vi "Change Database.vi"(8 "error in (no error)":errorcluster, 11 "Node Ptr":u64 format="%.0x") -> (0 "error out":errorcluster)   [LabVIEW 2025, in "Protection and Counter Addon System Explorer.lvlib"]
uses:
  Protection and Counter Addon System Explorer.lvlib
  Types/Database Changes VS Existing Frames.ctl
  Types/Base Frame Info.ctl
  <vilib>/NI VeriStand/Custom Device API/Custom Device Item Ref.ctl
  Types/CAN Filter Type.ctl
  Addon Shared/SubVIs/GUID Lookup.vi
  <vilib>/NI/NI VeriStand Advanced SysDef API/_SubVIs/SysDef.Search.GUIDs.vi
  <vilib>/NI VeriStand/Custom Device API/Get Item Property (U32).vi
  Addon Shared/Protection and Counter Addon Shared.lvlib
  <vilib>/NI/NI VeriStand Advanced SysDef API/SysDef API/Advanced System Definition.lvlib
  <vilib>/NI VeriStand/Custom Device API/Custom Device API.lvlib
  <resource>/objmgr/xnet.rc
  <vilib>/NI VeriStand/Custom Device Tools/Custom Device Utility Library/Custom Device Utility Library.lvlib
panel:
  in  "Tag":string
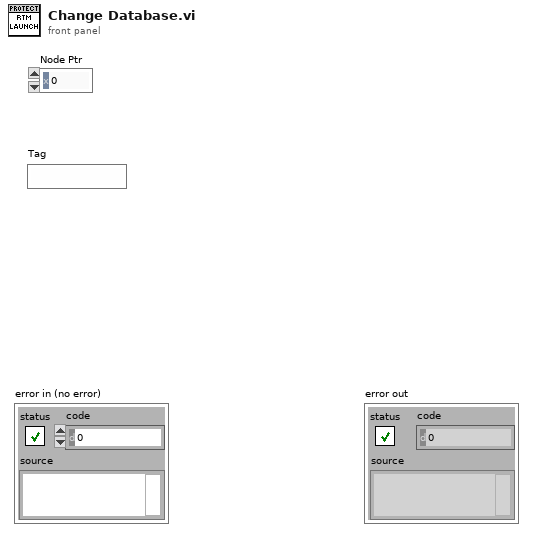
[diagram p1: front panel]
types:
  T1 = typedef "Protection and Counter Addon System Explorer.lvlib/Database Changes VS Existing Frames.ctl" = cluster{"Incoming":T2[], "Outgoing":T2[]}
  T2 = typedef "Protection and Counter Addon System Explorer.lvlib/Base Frame Info.ctl" = cluster{"Name":string, "ID":u32, "Signals":string[], "Node Ref":T3, "Type":T4}
  T3 = typedef "Custom Device API.lvlib/Custom Device Item Ref.ctl" = u64
  T4 = typedef "Protection and Counter Addon System Explorer.lvlib/CAN Filter Type.ctl" = enum16{"Cyclic Data", "Event Data", "Cyclic/Event", "All"}
  T5 = typedef "Custom Device API.lvlib/Custom Device Item Info.ctl" = cluster{"Name":string, "Is Channel":bool, "GUID":string, "Is Waveform":bool}
  T6 = typedef "Protection and Counter Addon Shared.lvlib/XNET Settings.ctl" = cluster{"Database":refnum<k21>, "Cluster":refnum<k21>, "Port":string, "Baud rate [Bd]":u64, "Termination":u32, "CAN I/O Mode":u32, "FD Baud rate [Bd]":u64, "Priority":i32, "Use Legacy":bool, "FD ISO Mode":u32, "Default Max Counter Value":dbl, "Default Protect Type":T7, "Include All Channels":bool}
  T7 = typedef "Protection and Counter Support Shared.lvlib/Protection Type.ctl" = enum16{"Arb ID + Bytes Checksum with Inversion", "Arb ID + Bytes CRC with Inversion", "Reversed Raw Signal Checksum with Inversion", "Concatenated Two's Compliment"}
  T8 = typedef "Protection and Counter Addon System Explorer.lvlib/CAN Update Results.ctl" = cluster{"New Cluster":refnum<k21>, "Incoming":T9, "Outgoing":T9}
  T9 = typedef "Protection and Counter Addon System Explorer.lvlib/VS Update List.ctl" = cluster{"Frames to Delete":T3[], "Frames to Add":T10[], "Frames to Update":T12[]}
  T10 = typedef "Protection and Counter Addon System Explorer.lvlib/Base Frame Info_NoVS.ctl" = cluster{"Name":string, "ID":u32, "Signals":T11[], "Type":T4}
  T11 = typedef "Protection and Counter Addon System Explorer.lvlib/Signal Attributes.ctl" = cluster{"Name":string, "Value Table":string, "Units":string}
  T12 = typedef "Protection and Counter Addon System Explorer.lvlib/CAN Frame Update Results.ctl" = cluster{"Node Ref":T3, "Name":string, "ID":u32, "New Signals":T11[], "Delete Signals":string[], "Type":T4, "Update Signals":T11[]}
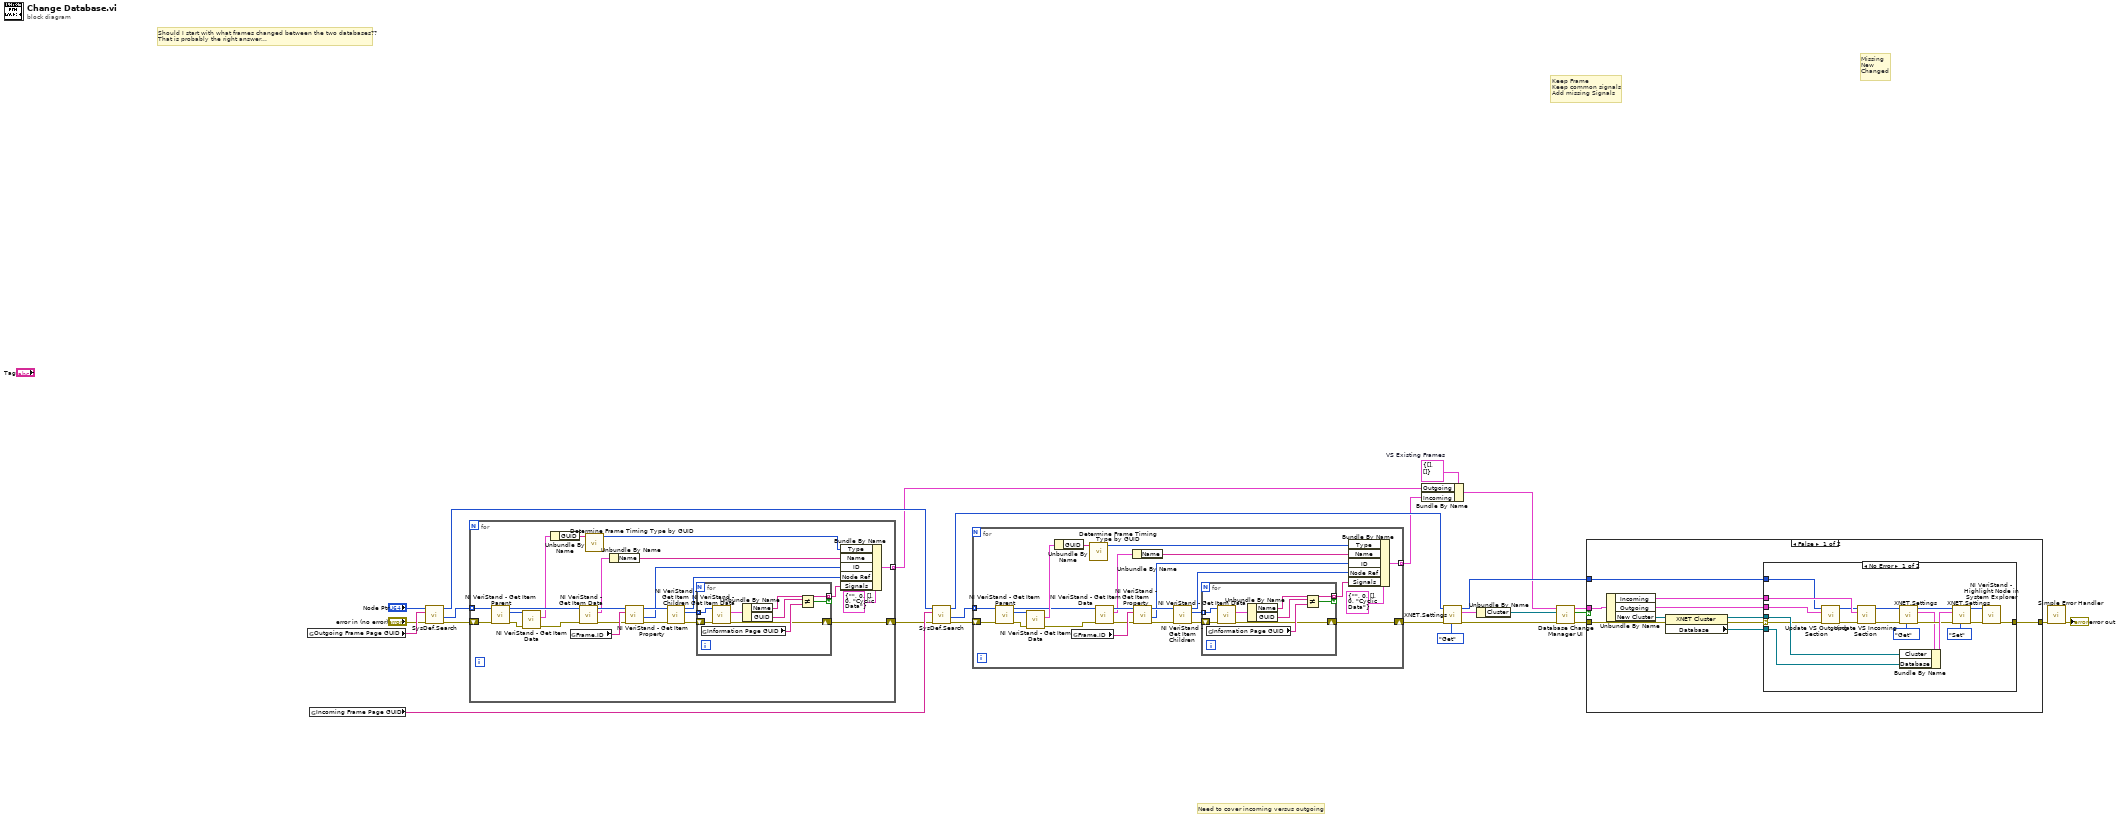
[diagram p0: block diagram]
diagram:
  w2 = T1 {"Incoming"=[], "Outgoing"=[]}  # VS Existing Frames
  # "Missing\nNew\nChanged"
  # "Should I start with what frames changed between the two databases??\nThat is probably the right answer..."
  # "Keep Frame\nKeep common signals\nAdd missing Signals"
  # "Need to cover incoming versus outgoing"
  n1 = global read "GUID Lookup.vi" "Outgoing Frame Page GUID"() -> (w26:string)
  n2 = global read "GUID Lookup.vi" "Incoming Frame Page GUID"() -> (w25:string)
  n3 = call-poly <vilib>:"SysDef.Search.vi"("error in (no error)"="error in (no error)", "GUID"=w26, "nodeID"="Node Ptr") -> ("error out"=w24:errorcluster, "Values Out"=w23:u64[], "nodeID out"=w19:u64)  [unwired: 5 in, 1 out]
  n4 = for {
    tunnel: w23 -> [w34] mode=indexing
    tunnel: [w40] -> w4 mode=indexing
    shift-right: [w39] -> w20
    shift-left: w24 -> [w33]
    n5 = call <vilib>:"NI VeriStand - Get Item Parent.vi"("error in (no error)"=w33, "Item Ref in"=w34) -> ("error out"=w31:errorcluster, "Parent Ref"=w32:T3, "Item Ref out"=w35:T3)  [unwired: 6 in, 1 out]
    n6 = call <vilib>:"NI VeriStand - Get Item Data.vi"("error in (no error)"=w31, "Item Ref in"=w32) -> ("error out"=w30:errorcluster, "Item Info"=w29:T5)  [unwired: 6 in, 2 out]
    n7 = Unbundle By Name(w29) -> ("GUID"=w28:string)
    n8 = global read "GUID Lookup.vi" "Frame.ID"() -> (w48:string)
    n9 = call <vilib>:"NI VeriStand - Get Item Data.vi"("error in (no error)"=w30, "Item Ref in"=w35) -> ("error out"=w45:errorcluster, "Item Info"=w43:T5, "Item Ref out"=w44:T3)  [unwired: 6 in, 1 out]
    n10 = call "Determine Frame Timing Type by GUID.vi"("GUID"=w28) -> ("CAN:Frame Type"=w27:T4)  [unwired: 10 in]
    n11 = Unbundle By Name(w43) -> ("Name"=w37:string)
    n12 = call-poly <vilib>:"NI VeriStand - Get Item Property.vi"("error in (no error)"=w45, "Property Name"=w48, "Item Ref in"=w44) -> ("error out"=w49:errorcluster, "Value"=w42:u32, "Item Ref out"=w50:T3)  [unwired: 5 in, 1 out]
    n13 = call <vilib>:"NI VeriStand - Get Item Children.vi"("error in (no error)"=w49, "Item Ref in"=w50) -> ("error out"=w46:errorcluster, "Child Refs"=w47:T3[], "Item Ref out"=w36:T3)  [unwired: 6 in, 1 out]
    n14 = for {
      tunnel: w47 -> [w58] mode=indexing
      shift-right: [w53] -> w39
      shift-left: w46 -> [w57]
      tunnel: [w51] -> w41 mode=indexing if=w52
      n15 = global read "GUID Lookup.vi" "Information Page GUID"() -> (w55:string)
      n16 = call <vilib>:"NI VeriStand - Get Item Data.vi"("error in (no error)"=w57, "Item Ref in"=w58) -> ("error out"=w53:errorcluster, "Item Info"=w56:T5)  [unwired: 6 in, 2 out]
      n17 = Unbundle By Name(w56) -> ("Name"=w51:string, "GUID"=w54:string)
      n18 = Not Equal?(x=w54, y=w55) -> (x != y?=w52:bool)
    }
    n19 = Bundle By Name(cluster=T2 {"Name"="", "ID"=0, "Signals"=[], "Node Ref"=0, "Type"=enum."Cyclic Data"}, "Type"=w27, "Name"=w37, "ID"=w42, "Node Ref"=w36, "Signals"=w41) -> (w40:T2)
  }
  n20 = call-poly <vilib>:"SysDef.Search.vi"("error in (no error)"=w20, "GUID"=w25, "nodeID"=w19) -> ("error out"=w21:errorcluster, "Values Out"=w22:u64[], "nodeID out"=w11:u64)  [unwired: 5 in, 1 out]
  n21 = for {
    tunnel: w22 -> [w62] mode=indexing
    shift-right: [w71] -> w12
    shift-left: w21 -> [w63]
    tunnel: [w70] -> w3 mode=indexing
    n22 = call <vilib>:"NI VeriStand - Get Item Parent.vi"("error in (no error)"=w63, "Item Ref in"=w62) -> ("error out"=w66:errorcluster, "Parent Ref"=w67:T3, "Item Ref out"=w60:T3)  [unwired: 6 in, 1 out]
    n23 = call <vilib>:"NI VeriStand - Get Item Data.vi"("error in (no error)"=w66, "Item Ref in"=w67) -> ("error out"=w61:errorcluster, "Item Info"=w65:T5)  [unwired: 6 in, 2 out]
    n24 = Unbundle By Name(w65) -> ("GUID"=w64:string)
    n25 = global read "GUID Lookup.vi" "Frame.ID"() -> (w80:string)
    n26 = call "Determine Frame Timing Type by GUID.vi"("GUID"=w64) -> ("CAN:Frame Type"=w59:T4)  [unwired: 10 in]
    n27 = call <vilib>:"NI VeriStand - Get Item Data.vi"("error in (no error)"=w61, "Item Ref in"=w60) -> ("error out"=w79:errorcluster, "Item Info"=w73:T5, "Item Ref out"=w77:T3)  [unwired: 6 in, 1 out]
    n28 = Unbundle By Name(w73) -> ("Name"=w72:string)
    n29 = call-poly <vilib>:"NI VeriStand - Get Item Property.vi"("error in (no error)"=w79, "Property Name"=w80, "Item Ref in"=w77) -> ("error out"=w78:errorcluster, "Value"=w74:u32, "Item Ref out"=w76:T3)  [unwired: 5 in, 1 out]
    n30 = call <vilib>:"NI VeriStand - Get Item Children.vi"("error in (no error)"=w78, "Item Ref in"=w76) -> ("error out"=w81:errorcluster, "Child Refs"=w82:T3[], "Item Ref out"=w68:T3)  [unwired: 6 in, 1 out]
    n31 = for {
      tunnel: w82 -> [w90] mode=indexing
      shift-right: [w85] -> w71
      shift-left: w81 -> [w89]
      tunnel: [w83] -> w75 mode=indexing if=w84
      n32 = global read "GUID Lookup.vi" "Information Page GUID"() -> (w87:string)
      n33 = call <vilib>:"NI VeriStand - Get Item Data.vi"("error in (no error)"=w89, "Item Ref in"=w90) -> ("error out"=w85:errorcluster, "Item Info"=w88:T5)  [unwired: 6 in, 2 out]
      n34 = Unbundle By Name(w88) -> ("Name"=w83:string, "GUID"=w86:string)
      n35 = Not Equal?(x=w86, y=w87) -> (x != y?=w84:bool)
    }
    n36 = Bundle By Name(cluster=T2 {"Name"="", "ID"=0, "Signals"=[], "Node Ref"=0, "Type"=enum."Cyclic Data"}, "Type"=w59, "Name"=w72, "ID"=w74, "Node Ref"=w68, "Signals"=w75) -> (w70:T2)
  }
  n37 = Bundle By Name(cluster=w2, "Outgoing"=w4, "Incoming"=w3) -> (w1:T1)
  n38 = call "XNET.Settings.vi"("Action"=enum8{"Get", "Set"}."Get", "error in (no error)"=w12, "Parent Ref in"=w11) -> ("error out"=w9:errorcluster, "XNET Settings"=w7:T6, "Item Ref out"=w6:T3)  [unwired: 6 in]
  n39 = Unbundle By Name(w7) -> ("Cluster"=w8:refnum<k21>)
  n40 = call "Database Change Manager UI.vi"("error in (no error)"=w9, "Old Cluster"=w8, "VS Existing Frames"=w1) -> ("error out"=w16:errorcluster, "Cancel Out"=w15:bool, "Change"=w14:T8)  [unwired: 6 in]
  n41 = case shown="False" w15 {
    tunnel: w16 -> [w94 w121]
    tunnel: w14 -> [w100 _]
    tunnel: [w91 w121] -> w13
    tunnel: w6 -> [w97 _]
    frame False {
      n42 = Unbundle By Name(w100) -> ("Incoming"=w93:T9, "Outgoing"=w95:T9, "New Cluster"=w96:refnum<k21>)
      n43 = property class="XNET Cluster"(reference=w96, error in=w94) -> (reference out=w99:refnum<k21>, error out=w92:errorcluster, "Database"=w98:refnum<k21>)
      n44 = case shown="No Error" w92 {
        selector: w92 -> [w114 w120]
        tunnel: w99 -> [w119 _]
        tunnel: w98 -> [w118 _]
        tunnel: w97 -> [w108 _]
        tunnel: w95 -> [w117 _]
        tunnel: [w107 w120] -> w91
        tunnel: w93 -> [w115 _]
        frame No Error {
          n45 = call "Update VS Outgoing Section.vi"("error in (no error)"=w114, "Outgoing"=w117, "Item Ref in"=w108) -> ("error out"=w116:errorcluster, "Item Ref out"=w113:T3)  [unwired: 7 in]
          n46 = call "Update VS Incoming Section.vi"("error in (no error)"=w116, "Outgoing"=w115, "Item Ref in"=w113) -> ("error out"=w105:errorcluster, "Item Ref out"=w103:T3)  [unwired: 7 in]
          n47 = call "XNET.Settings.vi"("Action"=enum8{"Get", "Set"}."Get", "error in (no error)"=w105, "Parent Ref in"=w103) -> ("error out"=w104:errorcluster, "XNET Settings"=w101:T6, "Item Ref out"=w102:T3)  [unwired: 6 in]
          n48 = Bundle By Name(cluster=w101, "Cluster"=w119, "Database"=w118) -> (w109:T6)
          n49 = call "XNET.Settings.vi"("Action"=enum8{"Get", "Set"}."Set", "error in (no error)"=w104, "XNET Settings"=w109, "Parent Ref in"=w102) -> ("error out"=w111:errorcluster, "Item Ref out"=w112:T3)  [unwired: 5 in, 1 out]
          n50 = call <vilib>:"NI VeriStand - Highlight Node in System Explorer.vi"("error in (no error)"=w111, "Item Ref in"=w112) -> ("error out"=w107:errorcluster)  [unwired: 8 in, 1 out]
        }
        frame Error {
        }
      }
    }
    frame True {
    }
  }
  n51 = call <vilib>:"Simple Error Handler.vi"("error in (no error)"=w13) -> ("error out"=→"error out":errorcluster)  [unwired: 4 in, 4 out]
